vi "Search_index_all.vi"(8 "error in (no error)":errorcluster caption="错误输入（无错误）", 11 "Procotol_class 输入":refnum<class "Procotol_class.lvclass">) -> (0 "error out":errorcluster caption="错误输出", 3 "Procotol_class 输出":refnum<class "Procotol_class.lvclass">)   [LabVIEW 2025, in "Procotol_class.lvclass"]
uses:
  Procotol_class.lvclass
  Procotol_class.lvclass/Procotol_class.ctl
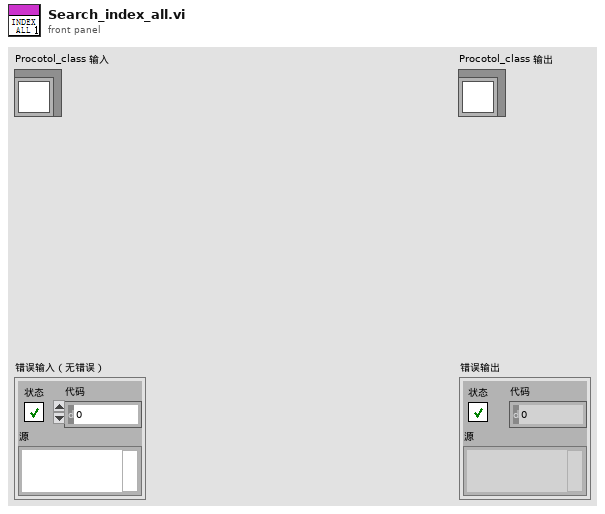
[diagram p1: front panel]
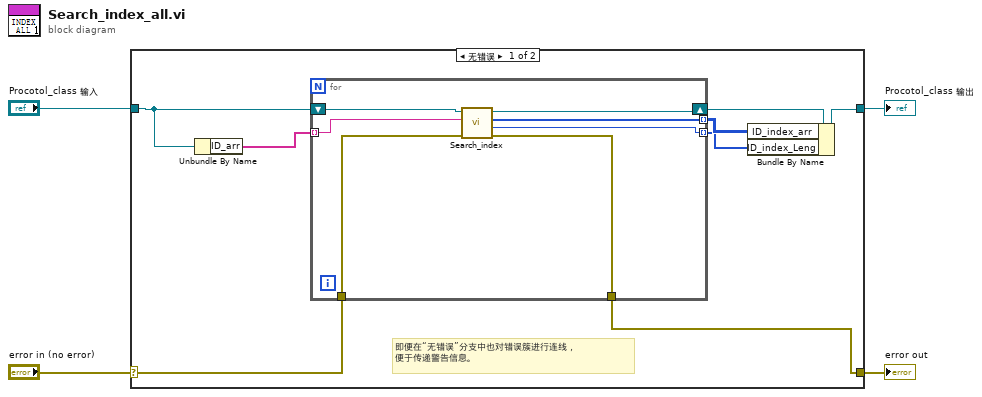
[diagram p0: block diagram]
diagram:
  n1 = case shown="无错误" "error in (no error)" {
    selector: "error in (no error)" -> [w12 w21]
    tunnel: [w11 w21] -> w3
    tunnel: [w9 w20] -> w1
    tunnel: "Procotol_class 输入" -> [w7 w20]
    frame No Error {
      # "即便在“无错误”分支中也对错误簇进行连线，\n便于传递警告信息。"
      n2 = Unbundle By Name(w7) -> ("ID_arr"=w6:string[])
      n3 = for {
        shift-right: [w18] -> w10
        shift-left: w7 -> [w19]
        tunnel: w12 -> [w17]
        tunnel: [w16] -> w11
        tunnel: w6 -> [w15] mode=indexing
        tunnel: [w14] -> w8 mode=indexing
        tunnel: [w13] -> w5 mode=indexing
        n4 = call-dynamic "Search_index.vi"("error in (no error)"=w17, "ID"=w15, "Procotol_class 输入"=w19) -> ("error out"=w16:errorcluster, "numb_index"=w13:i32, "ARR_index"=w14:i32[], "Procotol_class 输出"=w18:refnum<class "Procotol_class.lvclass">)  [unwired: 5 in]
      }
      n5 = Bundle By Name(cluster=w10, "ID_index_arr"=w8, "ID_index_Leng"=w5) -> (w9:refnum<class "Procotol_class.lvclass">)
    }
    frame Error {
    }
  }
  "error out" <- w3
  "Procotol_class 输出" <- w1
